vi "query ULRMC Modulation.vi"(8 "error in (no error)":errorcluster, 11 "NR in":refnum<class "NR.lvclass">) -> (0 "error out":errorcluster, 2 "Modulation":T1, 3 "NR out":refnum<class "NR.lvclass">)   [LabVIEW 2023, in "ANRITSU Call Box.lvlib" / "NR.lvclass"]
uses:
  NR.lvclass
  Type Definition/NR Modulation Type.ctl
  ANRITSU Call Box.lvlib
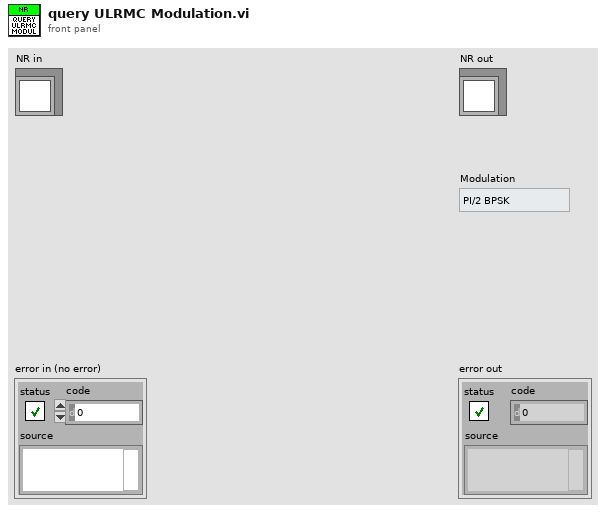
[diagram p1: front panel]
types:
  T1 = typedef "ANRITSU Call Box.lvlib/NR Modulation Type.ctl" = enum16{"PI/2 BPSK", "QPSK", "16QAM", "64QAM", "256QAM"}
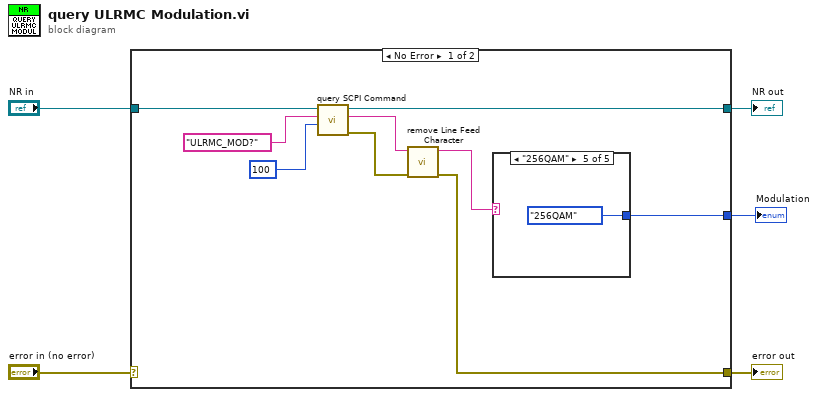
[diagram p0: block diagram]
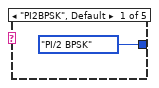
[diagram p2: hidden frame]
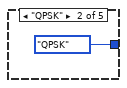
[diagram p3: hidden frame]
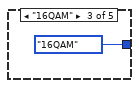
[diagram p4: hidden frame]
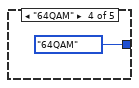
[diagram p5: hidden frame]
diagram:
  n1 = case shown="No Error" "error in (no error)" {
    selector: "error in (no error)" -> [_ w21]
    tunnel: [w6 w21] -> w4
    tunnel: [w9 w20] -> w2
    tunnel: "NR in" -> [w14 w20]
    tunnel: [w8 _] -> w1
    frame No Error {
      n2 = call "query SCPI Command.vi"("Read Buffer Length"=u32 100, "SCPI Command"="ULRMC_MOD?" ("initial string"), "NR in"=w14) -> ("error out"=w7:errorcluster, "Read Buffer String"=w11:string, "NR out"=w9:refnum<class "NR.lvclass">)  [unwired: 6 in]
      n3 = call "remove Line Feed Character.vi"("error in"=w7, "Query String"=w11) -> ("error out"=w6:errorcluster, "Line Feed Removed String"=w10:string)  [unwired: 8 in]
      n4 = case shown="\"256QAM\"" w10 {
        tunnel: [NR_Modulation_Type."PI/2 BPSK" ("Modulation 2") NR_Modulation_Type."QPSK" ("Modulation 2") NR_Modulation_Type."16QAM" ("Modulation 2") NR_Modulation_Type."64QAM" ("Modulation 2") NR_Modulation_Type."256QAM" ("Modulation 2")] -> w8
        frame "PI2BPSK", Default {
        }
        frame "QPSK" {
        }
        frame "16QAM" {
        }
        frame "64QAM" {
        }
        frame "256QAM" {
        }
      }
    }
    frame Error {
    }
  }
  "error out" <- w4
  "NR out" <- w2
  "Modulation" <- w1
